vi "VI_Tree_USBControl.vi"() -> ()   [LabVIEW 2013]
panel:
  in  "BMP file path":path
  out "HeadSerial":string
  out "CBTemp":dbl
  out "HeadTemp":dbl
  out "bID":u8
  # "Please check the block diagram."
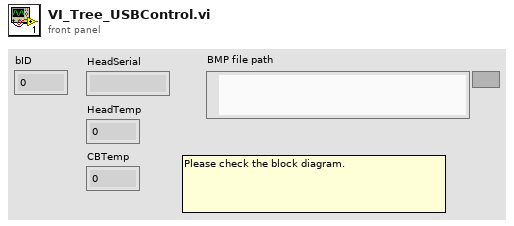
[diagram p1: front panel]
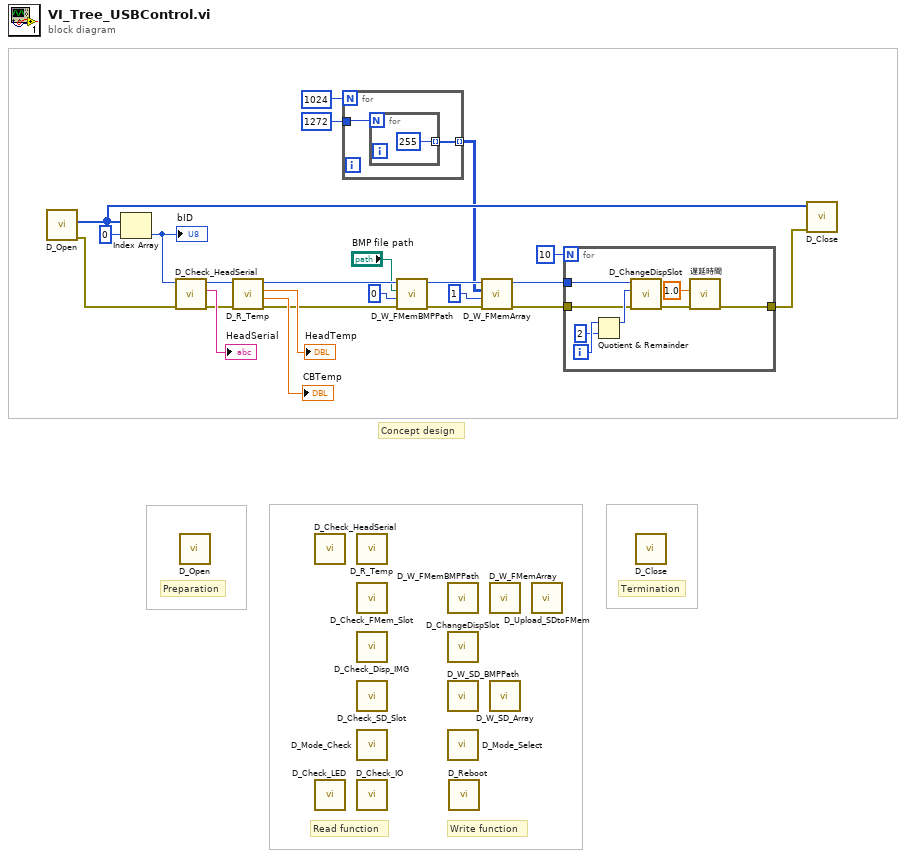
[diagram p0: block diagram]
diagram:
  # "Concept design"
  # "Write function"
  # "Read function"
  # "Termination"
  # "Preparation"
  n1 = call "D_Open.vi"() -> ("error out"=w5:errorcluster, "bIDList"=w22:u8[])  [unwired: 9 in, 1 out]
  n2 = Index Array(array=w22, index=0 ("指標")) -> (element=w20:u8)
  "bID" <- w20
  n3 = call "D_Check_HeadSerial.vi"("error in (no error)"=w5, "bID"=w20) -> ("error out"=w4:errorcluster, "HeadSerial"=→"HeadSerial":string, "bID"=w19:u8)  [unwired: 6 in, 1 out]
  n4 = call "D_Open.vi"() -> ()  [unwired: 9 in, 3 out]
  n5 = call "D_R_Temp.vi"("error in (no error)"=w4, "bID"=w19) -> ("error out"=w3:errorcluster, "CBTemp"=→"CBTemp":dbl, "HeadTemp"=→"HeadTemp":dbl, "bID"=w16:u8)  [unwired: 5 in, 1 out]
  n6 = call "D_Check_HeadSerial.vi"() -> ()  [unwired: 8 in, 4 out]
  n7 = call "D_Check_LED.vi"() -> ()  [unwired: 7 in, 5 out]
  n8 = for {
    N: 1024 -> [_]
    tunnel: 1272 -> [w25]
    tunnel: [w24] -> w8 mode=indexing
    n9 = for {
      N: w25 -> [_]
      tunnel: [u8 255] -> w24 mode=indexing
    }
  }
  n10 = call "D_R_Temp.vi"() -> ()  [unwired: 7 in, 5 out]
  n11 = call "D_Check_FMem_Slot.vi"() -> ()  [unwired: 8 in, 4 out]
  n12 = call "D_Check_Disp_IMG.vi"() -> ()  [unwired: 7 in, 5 out]
  n13 = call "D_Check_SD_Slot.vi"() -> ()  [unwired: 8 in, 4 out]
  n14 = call "D_Mode_Check.vi"() -> ()  [unwired: 8 in, 4 out]
  n15 = call "D_Check_IO.vi"() -> ()  [unwired: 7 in, 5 out]
  n16 = call "D_W_FMemBMPPath.vi"("error in (no error)"=w3, "slotNo"=u32 0, "BMP file path"="BMP file path", "bID"=w16) -> ("error out"=w2:errorcluster, "bID"=w15:u8)  [unwired: 5 in, 1 out]
  n17 = call "D_W_FMemBMPPath.vi"() -> ()  [unwired: 9 in, 3 out]
  n18 = call "D_ChangeDispSlot.vi"() -> ()  [unwired: 9 in, 3 out]
  n19 = call "D_W_SD_BMPPath.vi"() -> ()  [unwired: 9 in, 3 out]
  n20 = call "D_Mode_Select.vi"() -> ()  [unwired: 9 in, 3 out]
  n21 = call "D_Reboot.vi"() -> ()  [unwired: 10 in, 2 out]
  n22 = call "D_W_FMemArray.vi"("error in (no error)"=w2, "slotNo"=u32 1, "2D array"=w8, "bID"=w15) -> ("error out"=w1:errorcluster, "bID"=w13:u8)  [unwired: 5 in, 1 out]
  n23 = call "D_W_FMemArray.vi"() -> ()  [unwired: 9 in, 3 out]
  n24 = call "D_W_SD_Array.vi"() -> ()  [unwired: 9 in, 3 out]
  n25 = call "D_Upload_SDtoFMem.vi"() -> ()  [unwired: 9 in, 3 out]
  n26 = for {
    N: 10 -> [_]
    tunnel: w13 -> [w34]
    tunnel: [w31] -> w6
    tunnel: w1 -> [w27]
    i -> [w30]
    n27 = Quotient & Remainder(x=w30, y=2) -> (x-y*floor(x/y)=w28:i32)  [unwired: 1 out]
    n28 = call "D_ChangeDispSlot.vi"("error in (no error)"=w27, "slotNo"=w28, "bID"=w34) -> ("error out"=w33:errorcluster)  [unwired: 6 in, 2 out]
    n29 = call "遅延時間"("error in (no error)"=w33, "Delay Time (s)"=1.0) -> ("error out"=w31:errorcluster)  [unwired: 9 in]
  }
  n30 = call "D_Close.vi"() -> ()  [unwired: 10 in, 2 out]
  n31 = call "D_Close.vi"("error in (no error)"=w6, "bIDList"=w22) -> ()  [unwired: 8 in, 2 out]
